vi "Delete_Table.vi"(8 "error in (no error)":errorcluster caption="错误输入（无错误）", 10 "table":string, 11 "Database_access 输入":refnum<class "Database_access.lvclass">) -> (0 "error out":errorcluster caption="错误输出", 3 "Database_access 输出":refnum<class "Database_access.lvclass">)   [LabVIEW 2025, in "Database_access.lvclass"]
uses:
  Database_access.lvclass
  Database_access.lvclass/Database_access.ctl
  <vilib>/addons/database/NI_Database_API.lvlib
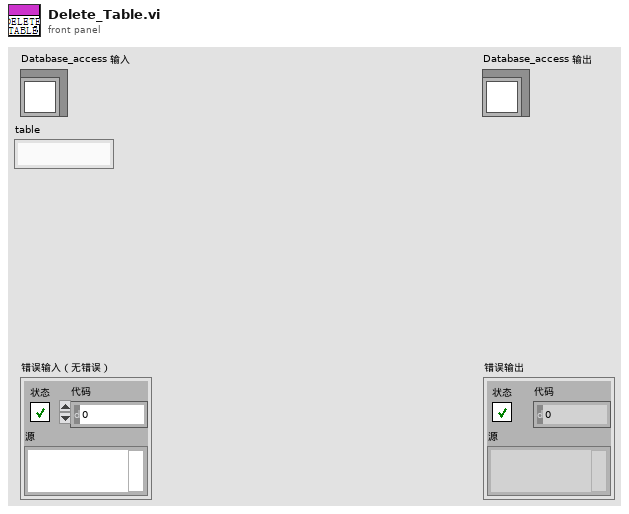
[diagram p1: front panel]
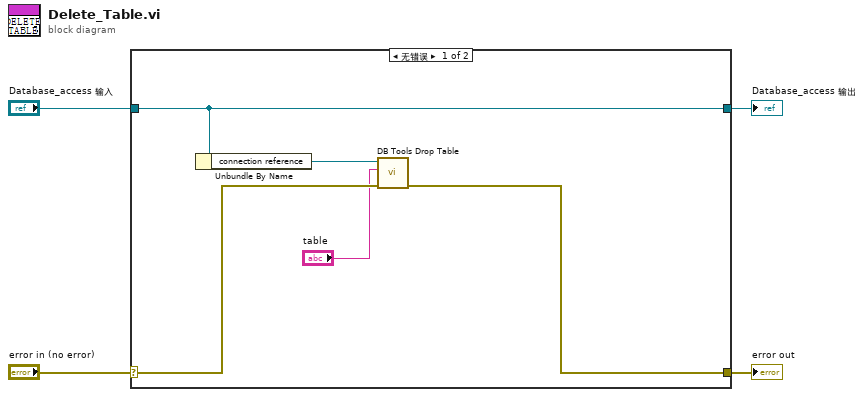
[diagram p0: block diagram]
diagram:
  n1 = case shown="无错误" "error in (no error)" {
    selector: "error in (no error)" -> [w7 w11]
    tunnel: [w6 w11] -> w3
    tunnel: [w9 w10] -> w1
    tunnel: "Database_access 输入" -> [w9 w10]
    frame No Error {
      n2 = Unbundle By Name(w9) -> ("connection reference"=w8:refnum<k1>)
      n3 = call <vilib>:"DB Tools Drop Table.vi"("error in (no error)"=w7, "table"="table", "connection reference"=w8) -> ("error out"=w6:errorcluster)  [unwired: 5 in, 1 out]
    }
    frame Error {
    }
  }
  "error out" <- w3
  "Database_access 输出" <- w1
